vi "Smart IO Initialize Mode.vi"(8 "error in (no error)":errorcluster, 9 "force":bool, 10 "mode":T1 items=["Digital Input"=0, "Digital Output"=1, "Analog Input"=2, "PWM Input"=3, "PWM Output"=4, "Counter Rising"=5, "Counter Falling"=6, "Quadrature"=7, "Addressable LEDs"=13], 11 "deviceIndex":i32=-1) -> (0 "error out":errorcluster)   [LabVIEW 2023, in "MrcLib.lvlib"]
doc: "Configures the indicated device channel for a specific mode of I/O operation."
uses:
  <vilib>/MRC/MrcLib.lvlib
  <vilib>/MRC/Types/MRC Smart IO Mode.ctl
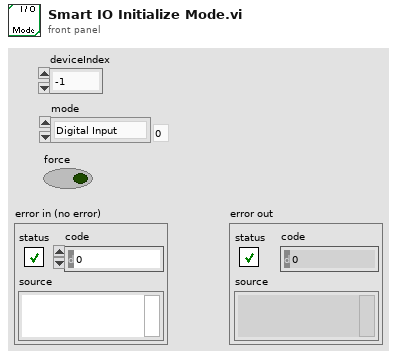
[diagram p1: front panel]
types:
  T1 = typedef "MRC Smart IO Mode.ctl" = i32
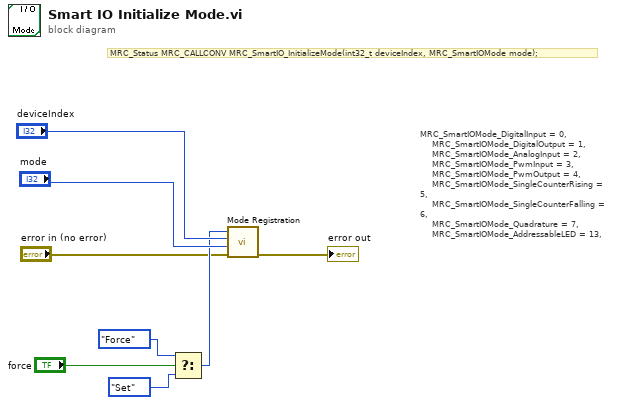
[diagram p0: block diagram]
diagram:
  # "MRC_SmartIOMode_DigitalInput = 0,\n    MRC_SmartIOMode_DigitalOutput = 1,\n    MRC_SmartIOMode_AnalogInput = 2,\n    MRC_SmartIOMode_PwmInput = 3,\n    MRC_SmartIOMode_PwmOutput = 4,\n    MRC_SmartIOMode_SingleCounterRising = 5,\n    MRC_SmartIOMode_SingleCounterFalling = 6,\n    MRC_SmartIOMode_Quadrature = 7,\n    MRC_SmartIOMode_AddressableLED = 13,"
  # "MRC_Status MRC_CALLCONV MRC_SmartIO_InitializeMode(int32_t deviceIndex, MRC_SmartIOMode mode);"
  n1 = Select(t=enum16{"Get", "Set", "Force", "Clear"}."Force" ("Action"), s="force", f=enum16{"Get", "Set", "Force", "Clear"}."Set" ("Action")) -> (s? t:f=w3:enum16{"Get", "Set", "Force", "Clear"})
  n2 = call <vilib>:"Mode Registration.vi"("error in"="error in (no error)", "mode"="mode", "device ID"="deviceIndex", "Action"=w3) -> ("error out"=→"error out":errorcluster)  [unwired: 6 in, 1 out]
